vi "Launch.vi"(8 "error in (no error)":errorcluster, 10 "NavigatorEvents":T1, 11 "View in":refnum<class "View.lvclass">) -> (0 "error out":errorcluster, 2 "VIReference":refnum<vi>, 3 "View out":refnum<class "View.lvclass">)   [LabVIEW 2024, in "Page1.lvlib" / "View.lvclass"]
doc: "Create stop event and launch view asynchronously.\n\nNavigatorEvents - used to navigate the app from inside a view's viewmodel. Do this by generating the relevant event (go, push, pop) and if necessary, pass in the route name (setup when Navigator is initialised).\n\nVIReference - this should output the VI reference of the view (UI) that has been launched. To launch a view, wire up the following: strictly typed Static VI Reference > Property Node (VI Path) > Open VI Reference > Start Asynchronous Call"
uses:
  View.lvclass
  Navigator/NavigatorEvents.ctl
  View.lvclass/View.ctl
  UI.vi
  NavigatableView/NavigatableView.lvclass
  Navigator/Navigator.lvclass
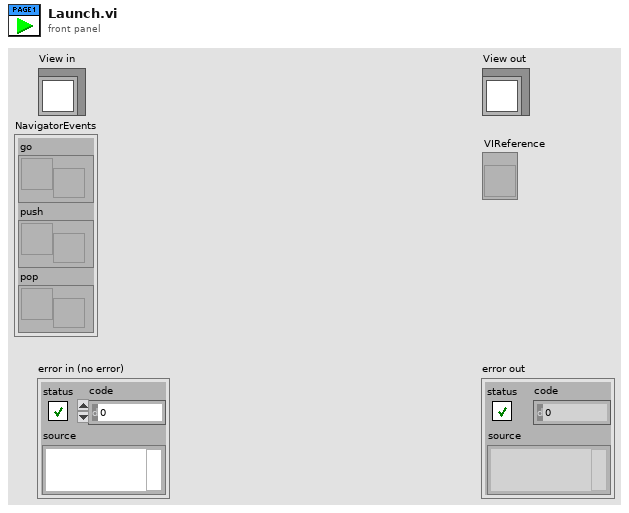
[diagram p1: front panel]
types:
  T1 = typedef "Navigator.lvclass/NavigatorEvents.ctl" = cluster{"go":refnum<user-event>, "push":refnum<user-event>, "pop":refnum<user-event>}
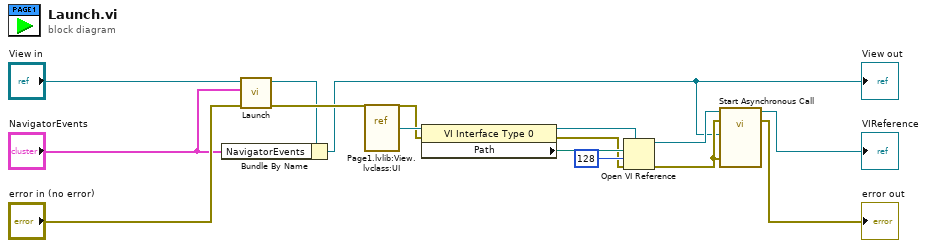
[diagram p0: block diagram]
diagram:
  n1 = call-parent "Launch.vi"("error in (no error)"="error in (no error)", "NavigatorEvents"="NavigatorEvents", "NavigatableView in"="View in") -> ("error out"=w6:errorcluster, "NavigatableView out"=w3:refnum<class "View.lvclass">)  [unwired: 6 in, 1 out]
  n2 = Bundle By Name(cluster=w3, "NavigatorEvents"="NavigatorEvents") -> (w1:refnum<class "View.lvclass">)
  "View out" <- w1
  n3 = vi-ref "Page1.lvlib:View.lvclass:UI.vi"() -> (w7:refnum<vi>)
  n4 = property class="VI Interface Type 0"(reference=w7, error in=w6) -> (reference out=w10:refnum<vi>, error out=w9:errorcluster, "Path"=w13:path)
  n5 = Open VI Reference(type specifier VI Refnum (for type only)=w10, vi path=w13, options=128, error in (no error)=w9) -> (vi reference=w8:refnum<vi>, error out=w11:errorcluster)  [unwired: 2 in]
  n6 = call-by-ref "Start Asynchronous Call"(reference=w8, error in=w11, 8:"error in (no error)"=w11, "View in"=w1) -> (reference out=→"VIReference":refnum<vi>, error out=→"error out":errorcluster)  [unwired: 8 in, 2 out]
